vi "Im the Bearer.vi"(8 "error in (no error)":errorcluster, 11 "Guardian in":refnum<class "Guardian.lvclass">) -> (0 "error out":errorcluster, 2 "I'm the Bearer":bool, 3 "Guardian out":refnum<class "Guardian.lvclass">)   [LabVIEW 2020, in "TALOS.lvlib" / "Guardian.lvlib" / "Guardian.lvclass"]
uses:
  Guardian.lvclass
  Guardian.lvclass/Guardian.ctl
  Ancestor/Ancestor/Ancestor.lvclass
  C:/Users/marco/Documents/GitHub_Lab/TALOS/talos/Ancestor/Ancestor/Ancestor.lvclass
  C:/Users/marco/Documents/GitHub_Lab/TALOS/builds/Actor Framework PPL/Actor Framework.lvlibp/1abvi3w/vi.lib/ActorFramework/Actor/Actor.lvclass
  C:/Users/marco/Documents/GitHub_Lab/TALOS/talos/Guardian/Guardian/Guardian.lvclass
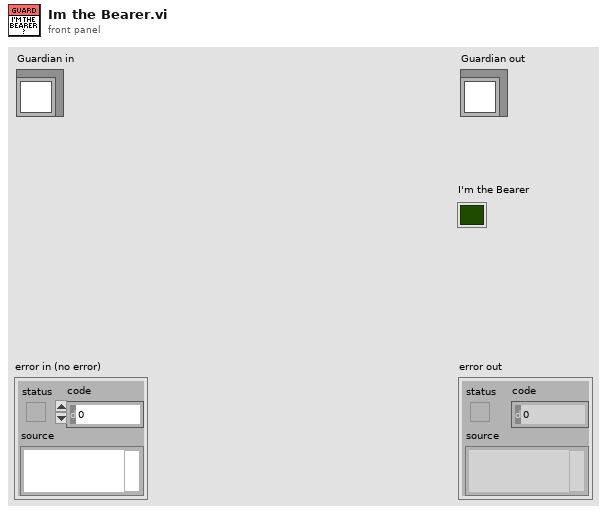
[diagram p1: front panel]
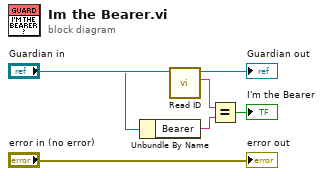
[diagram p0: block diagram]
diagram:
  n1 = call "Read ID.vi"("Ancestor in"="Guardian in") -> ("ID"=w3:string, "Ancestor out"=w4:refnum<class "Guardian.lvclass">)  [unwired: 8 in, 1 out]
  "Guardian out" <- w4
  n2 = Unbundle By Name(w4) -> ("Bearer"=w2:string)
  n3 = Equal?(x=w3, y=w2) -> (x = y?=→"I'm the Bearer":bool)
  "error out" <- "error in (no error)"
